vi "Init Msg Input.vi"(6 "Teller":refnum<class "Teller.lvclass">) -> (2 "Msg Input":refnum<class "Msg Input.lvclass">)   [LabVIEW 2020, in "_Template.lvlib" / "Templates.lvlib" / "TEMPLATE jettl Msg.lvlib" / "TEMPLATE Msg Input.lvlib"]
uses:
  TEMPLATE Msg Input.lvlib
  jettl/jettl/Msg Input/Msg Input.lvclass
  jettl/jettl/Teller/Teller.lvclass
  TEMPLATE Msg Input/TEMPLATE Msg Input.lvclass/TEMPLATE Msg Input.ctl
  TEMPLATE Msg Input/TEMPLATE Msg Input.lvclass
  C:/git/jettl/src/jettl/jettl/Msg Input/Msg Input.lvclass
panel:
  # "This front panel should not be manipulated."
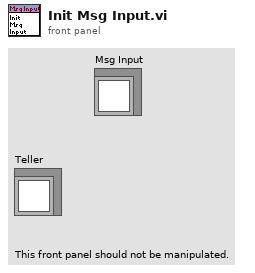
[diagram p1: front panel]
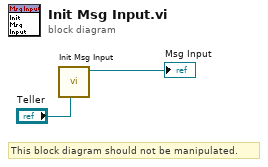
[diagram p0: block diagram]
diagram:
  # "This block diagram should not be manipulated."
  n1 = call "Init Msg Input.vi"("Teller"="Teller") -> ("TEMPLATE Msg Input out"=→"Msg Input":refnum<class "TEMPLATE Msg Input.lvclass">)  [unwired: 10 in]
